vi "Tree_Go to next displayed item.vi"(6 "Allow selection of disabled elements":bool, 7 "Direction":enum16{"Down", "Up"}(ring), 8 "error in (no error)":errorcluster, 11 "Tree ref":refnum<vi>) -> (0 "error out":errorcluster, 2 "discard":bool, 3 "Tree ref out":refnum<vi>)   [LabVIEW 2023]
doc: "Allow cycling on linstbox with key navigfation by determining if the curent selection is the first or last in the listbox and going to the last or first item if the up or dawn arrow (respectively) are pressed.\n\nUse the discard output to discard up and down arrow keys for functaions handled by this VI. Otherwise, allow the normal key functions to take place."
panel:
  out "first item":bool
  out "last item":bool
  in  "Tree":string[](tree)
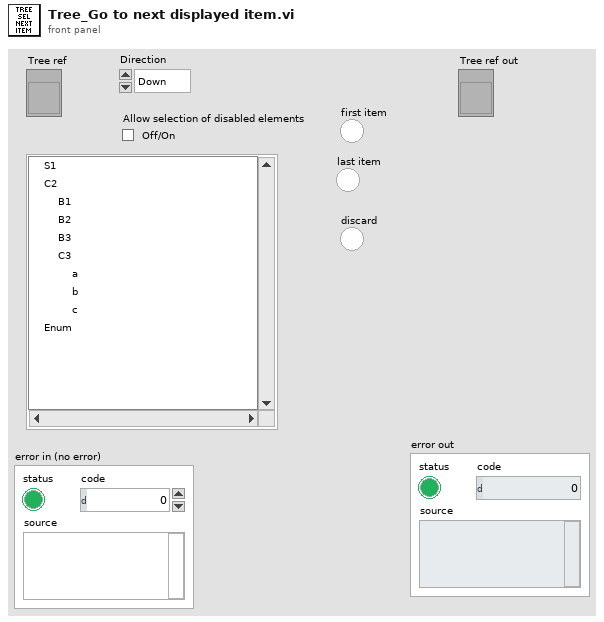
[diagram p1: front panel]
types:
  T1 = enum16{"Unknown", "Base", "Scripting", "Private", "Deprecated", "None", "Divider"}
  T2 = cluster{"Index":u16, "Property Type":enum16{"Unknown", "Base", "Scripting", "Private", "Deprecated", "None", "Divider"}, "ID String":string, "Dotted ID String":string, "Class":string, "Parent":string, "Display name full":string, "Display name short":string, "Parents Array":string[], "Indent":u16}
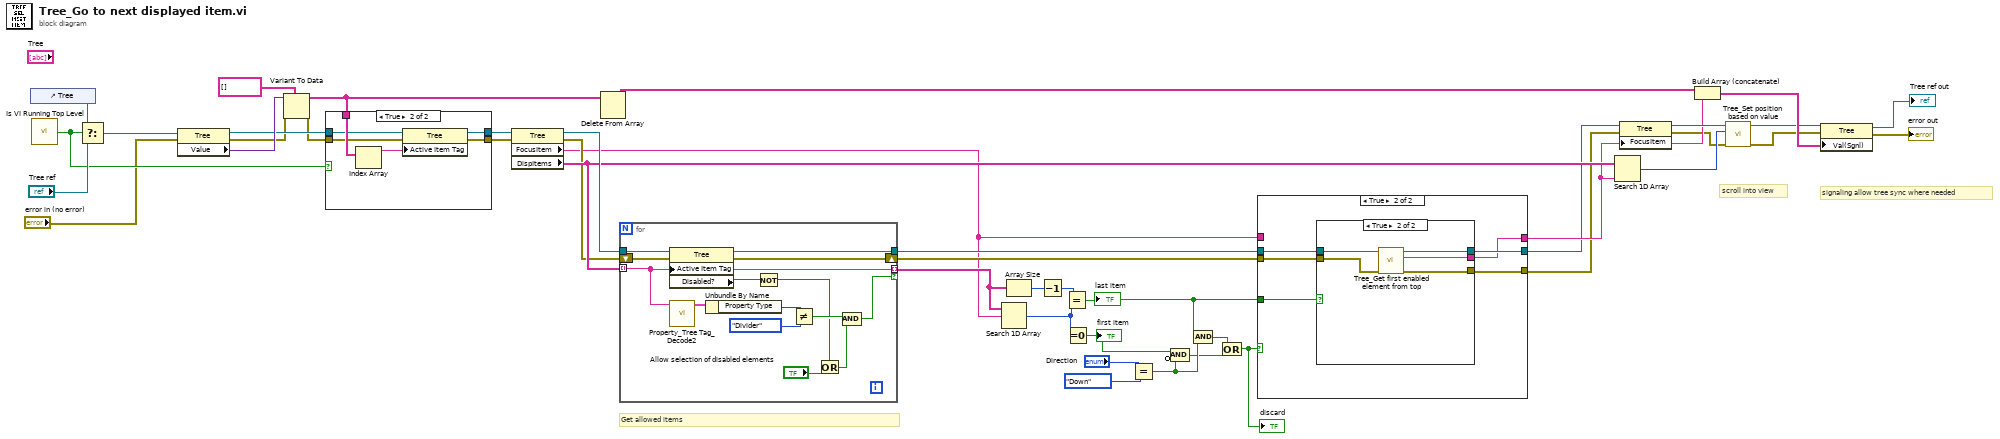
[diagram p0: block diagram]
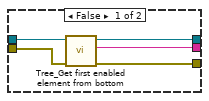
[diagram p4: hidden frame]
diagram:
  # "signaling allow tree sync where needed"
  # "scroll into view"
  # "Get allowed items"
  n1 = control-ref of="Tree"() -> (w43:refnum<vi>)
  n2 = call "Is VI Running Top Level.vi"() -> ("Top Level?"=w29:bool)  [unwired: 5 in]
  n3 = Select(t=w43, s=w29, f="Tree ref") -> (s? t:f=w35:refnum<vi>)
  n4 = property class="Tree"(reference=w35, error in="error in (no error)") -> (reference out=w31:refnum<vi>, error out=w14:errorcluster, "Value"=w32:variant)
  n5 = Variant To Data(error in=w14, type=string[] [] ("Active Item:Tag"), Variant=w32) -> (data=w34:string[], error out=w13:errorcluster)
  n6 = case shown="True" w29 {
    tunnel: w34 -> [_ w51]
    tunnel: w31 -> [w45 w49]
    tunnel: [w45 w48] -> w30
    tunnel: w13 -> [w44 w47]
    tunnel: [w44 w46] -> w12
    frame False {
    }
    frame True {
      n7 = Index Array(array=w51) -> (element=w50:string)  [unwired: 1 in]
      n8 = property class="Tree"(reference=w49, error in=w47, "Active Item Tag"=w50) -> (reference out=w48:refnum<vi>, error out=w46:errorcluster)
    }
  }
  n9 = property class="Tree"(reference=w30, error in=w12) -> (reference out=w37:refnum<vi>, error out=w10:errorcluster, "FocusItem"=w2:string, "DispItems"=w26:string[])
  n10 = Delete From Array(array=w34) -> (array with subset deleted=w38:string[])  [unwired: 2 in, 1 out]
  n11 = for {
    tunnel: w37 -> [w65]
    tunnel: [w64] -> w36 mode=indexing if=w58
    tunnel: w26 -> [w64] mode=indexing
    tunnel: [w60] -> w9
    shift-right: [w53] -> w7
    shift-left: w10 -> [w54]
    n12 = property class="Tree"(reference=w65, error in=w54, "Active Item Tag"=w64) -> (reference out=w60:refnum<vi>, error out=w53:errorcluster, "Disabled?"=w56:bool)
    n13 = call "Property_Tree Tag_Decode2.vi"("Tag In"=w64) -> ("TagData"=w63:T2)  [unwired: 10 in]
    n14 = Unbundle By Name(w63) -> ("Property Type"=w62:T1)
    n15 = Not(x=w56) -> (.not. x?=w52:bool)
    n16 = Not Equal?(x=w62, y=T1."Divider" ("Property Type")) -> (x != y?=w59:bool)
    n17 = Or(x=w52, y="Allow selection of disabled elements") -> (x .or. y?=w55:bool)
    n18 = Compound Arithmetic op=AND(w59, w55) -> (w58:bool)
  }
  n19 = Search 1D Array(1D array=w36, element=w2) -> (index of element=w18:i32)  [unwired: 1 in]
  n20 = Array Size(array=w36) -> (size(s)=w20:i32)
  n21 = Decrement(x=w20) -> (x-1=w19:i32)
  n22 = Equal?(x=w19, y=w18) -> (x = y?=w1:bool)
  "last item" <- w1
  n23 = Equal To 0?(x=w18) -> (x = 0?=w17:bool)
  "first item" <- w17
  n24 = Equal?(x="Direction", y=enum16{"Down", "Up"}."Down" ("Direction")) -> (x = y?=w16:bool)
  n25 = Compound Arithmetic op=AND(w17, invert w16) -> (w15:bool)
  n26 = Compound Arithmetic op=AND(w1, w16) -> (w3:bool)
  n27 = Compound Arithmetic op=OR(w3, w15) -> (w5:bool)
  "discard" <- w5
  n28 = case shown="True" w5 {
    tunnel: [w66 w70] -> w25
    tunnel: w9 -> [w68 w74]
    tunnel: [w68 w73] -> w8
    tunnel: w7 -> [w67 w72]
    tunnel: [w67 w71] -> w6
    tunnel: w2 -> [w66 _]
    tunnel: w1 -> [_ w69]
    frame False {
    }
    frame True {
      n29 = case shown="True" w69 {
        tunnel: w74 -> [w79 w84]
        tunnel: [w78 w83] -> w73
        tunnel: w72 -> [w77 w81]
        tunnel: [w76 w82] -> w71
        tunnel: [w75 w80] -> w70
        frame False {
          n30 = call "Tree_Get first enabled element from bottom.vi"("error in (no error)"=w77, "TreeControl Ref"=w79) -> ("error out"=w76:errorcluster, "First Element Tag"=w75:string, "Tree Control Ref Out"=w78:refnum<vi>)  [unwired: 7 in]
        }
        frame True {
          n31 = call "Tree_Get first enabled element from top.vi"("error in (no error)"=w81, "Tree Control Ref"=w84) -> ("error out"=w82:errorcluster, "First Enabled Element"=w80:string, "Tree Control Ref Out"=w83:refnum<vi>)  [unwired: 7 in]
        }
      }
    }
  }
  n32 = Search 1D Array(1D array=w26, element=w25) -> (index of element=w24:i32)  [unwired: 1 in]
  n33 = property class="Tree"(reference=w8, error in=w6, "FocusItem"=w25) -> (reference out=w28:refnum<vi>, error out=w23:errorcluster)
  n34 = Build Array (concatenate)(w38, w25) -> (w39:string[])
  n35 = call "Tree_Set position based on value.vi"("error in (no error)"=w23, "Selected Row"=w24, "Tree Ref"=w28) -> ("error out"=w22:errorcluster, "Tree Ref"=w27:refnum<vi>)  [unwired: 7 in]
  n36 = property class="Tree"(reference=w27, error in=w22, "Val(Sgnl)"=w39) -> (reference out=→"Tree ref out":refnum<vi>, error out=→"error out":errorcluster)
